vi "Pre Launch Init.vi"(11 "WebSocket Client in":refnum<class "WebSocket Client.lvclass">) -> (0 "error out":errorcluster, 3 "WebSocket Client out":refnum<class "WebSocket Client.lvclass">)   [LabVIEW 2021, in "WebSocket Actors.lvlib" / "WebSocket Client.lvclass"]
doc: "(<B>Filename</B>: Actor Framework.lvlib:Actor.lvclass:Pre Launch Init.vi)\n\nDefines behavior that occurs after the Launch Nested Actor method is invoked but before the actor's Actor Core method begins running.\n\nBy default, this method does nothing. A descendant class may override it to define behavior."
uses:
  WebSocket Client.lvclass
  C:/Projects/WebSocket-Actor/WebSocket Actor/WebSocket Connection/WebSocket Connection.lvclass
  WebSocket Client.lvclass/WebSocket Client.ctl
  WebSocket Connection/WebSocket Connection.lvclass/WebSocket Connection.ctl
  WebSocket Connection/properties/Read Timeout (ms).vi
  WebSocket Connection/properties/Write WebSocket Connection.vi
  WebSocket Connection/properties/Write Peer ID.vi
  WebSocket Connection/WebSocket Connection.lvclass
  <vilib>/LS Instruments AG/LV-WebSockets/LV WebSockets.lvlib
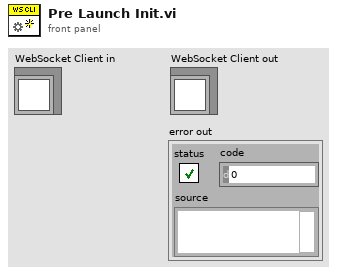
[diagram p1: front panel]
types:
  T1 = typedef "LV WebSockets.lvlib/Headers.ctl" = cluster{"Name":string, "Value":string}
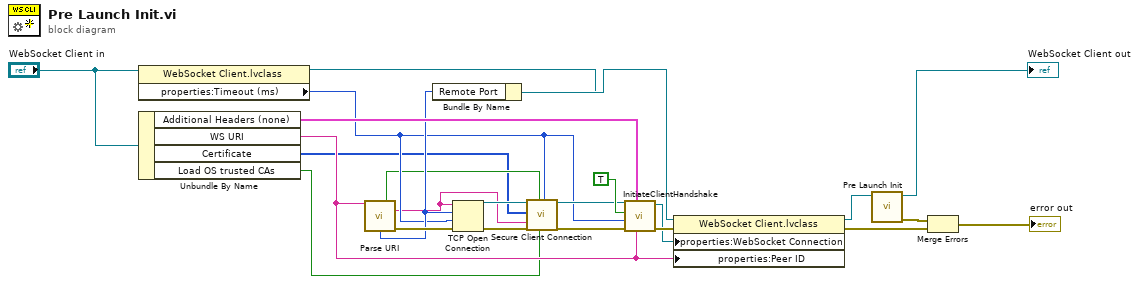
[diagram p0: block diagram]
diagram:
  n1 = property class="WebSocket Client.lvclass"(reference="WebSocket Client in") -> (reference out=w13:refnum<class "WebSocket Client.lvclass">, "properties:Timeout (ms)"=w6:i32)  [unwired: 1 in, 1 out]
  n2 = Unbundle By Name("WebSocket Client in") -> ("Additional Headers (none)"=w22:T1[], "WS URI"=w12:string, "Certificate"=w4:u8[], "Load OS trusted CAs"=w3:bool)
  n3 = call <vilib>:"Parse URI.vi"("URI"=w12) -> ("Secure"=w5:bool, "Hostname"=w1:string, "Port"=w14:u16, "error out"=w17:errorcluster)  [unwired: 7 in, 4 out]
  n4 = Bundle By Name(cluster=w13, "Remote Port"=w14) -> (w16:refnum<class "WebSocket Client.lvclass">)
  n5 = TCP Open Connection(address=w1, remote port or service name=w14, timeout ms (60000)=w6, error in (no error)=w17) -> (connection ID=w7:refnum<k5>, error out=w10:errorcluster)  [unwired: 1 in]
  n6 = call <vilib>:"Secure Client Connection.vi"("TCP connection"=w7, "certificate"=w4, "server hostname"=w1, "error in"=w10, "Secure the Connection (T)"=w5, "load OS trusted CAs?"=w3, "timeout (25000 ms)"=w6) -> ("TCP connection out"=w8:refnum<k5>, "error out"=w9:errorcluster)  [unwired: 10 in, 1 out]
  n7 = call <vilib>:"InitiateClientHandshake.vi"("WS URI"=w12, "additional headers (none)"=w22, "error in (no error)"=w9, "timeout ms (5000)"=w6, "Relative URI Request (F)"=TRUE, "WebSocket Connection in"=w8) -> ("error out"=w20:errorcluster, "WebSocket Connection out"=w11:refnum<k5>)  [unwired: 3 in, 1 out]
  n8 = property class="WebSocket Client.lvclass"(reference=w16, error in=w20, "properties:WebSocket Connection"=w11, "properties:Peer ID"=w12) -> (reference out=w21:refnum<class "WebSocket Client.lvclass">, error out=w18:errorcluster)
  n9 = call-parent "Pre Launch Init.vi"("Actor in"=w21) -> ("error out"=w24:errorcluster, "Actor out"=→"WebSocket Client out":refnum<class "WebSocket Client.lvclass">)  [unwired: 9 in]
  n10 = Merge Errors(w24, w18) -> (→"error out":errorcluster)
